vi "Load LV_data Values.vi"() -> ()   [LabVIEW 2020]
panel:
  out "array2_name 2":T1(array[cluster])=[[{"my_name"=45.6, "my_name2"=-12, "my_bool_array"=[TRUE], "Array"=[]}]]
  out "text":string
  in  "file path (use dialog)":path
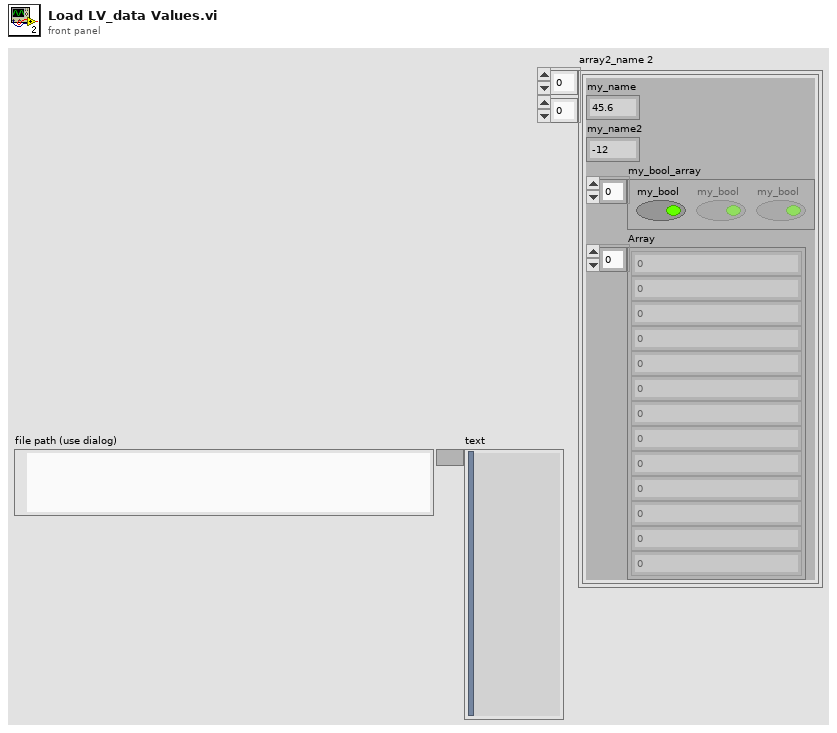
[diagram p1: front panel]
types:
  T1 = cluster{"my_name":dbl, "my_name2":i32, "my_bool_array":bool[], "Array":cdb[]}[][]
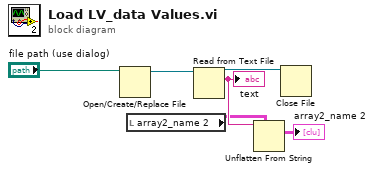
[diagram p0: block diagram]
diagram:
  n1 = Open/Create/Replace File(file path (use dialog)="file path (use dialog)") -> (refnum out=w5:refnum<file>)  [unwired: 5 in, 2 out]
  n2 = local read "array2_name 2"() -> (w2:T1)
  n3 = Read from Text File(file (use dialog)=w5) -> (refnum out=w4:refnum<file>, text=w3:string)  [unwired: 3 in, 2 out]
  "text" <- w3
  n4 = Unflatten From String(type=w2, binary string=w3) -> (value=→"array2_name 2":T1)  [unwired: 3 in, 2 out]
  n5 = Close File(refnum=w4) -> ()  [unwired: 1 in, 2 out]
